vi "Valid Path.vi"   [LabVIEW 2020, in "openg_file.lvlib"]
doc: "This polymorphic VI checks whether path (or array of paths) is valid, meaning not \"Empty path\" and not \"Not a Path\"."
uses:
  openg_file.lvlib
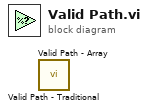
[diagram p0: block diagram]
diagram:
  n1 = call "Valid Path - Traditional.vi"() -> ()  [unwired: 1 in, 1 out]
  n2 = call "Valid Path - Array.vi"() -> ()  [unwired: 1 in, 1 out]
